vi "RemoteVI Status Convert.vi"(0 "raw":T2(array[cluster]), 1 "now":dbl) -> (4 "status":T1(array[cluster]))   [LabVIEW 2020, in "RemoteVI.lvlib"]
doc: "Turns the entries of RemoteVI Status Registry.vi into the status RemoteVI Status.vi returns, for the time now (seconds since the LabVIEW epoch): running is TRUE while the server loop published within the last 2 s; uptime s = now - started; per client connected s = now - since and idle s = now - last input, or -1 when the client sent no input yet; kB per s = bytes per s / 1024; hWnd (the shared window) is passed on. Pure function, cannot fail. Reference: statusConvert() in tools\\lib\\status.mjs, vectors tests\\vectors\\status.json (convert)."
uses:
  RemoteVI.lvlib
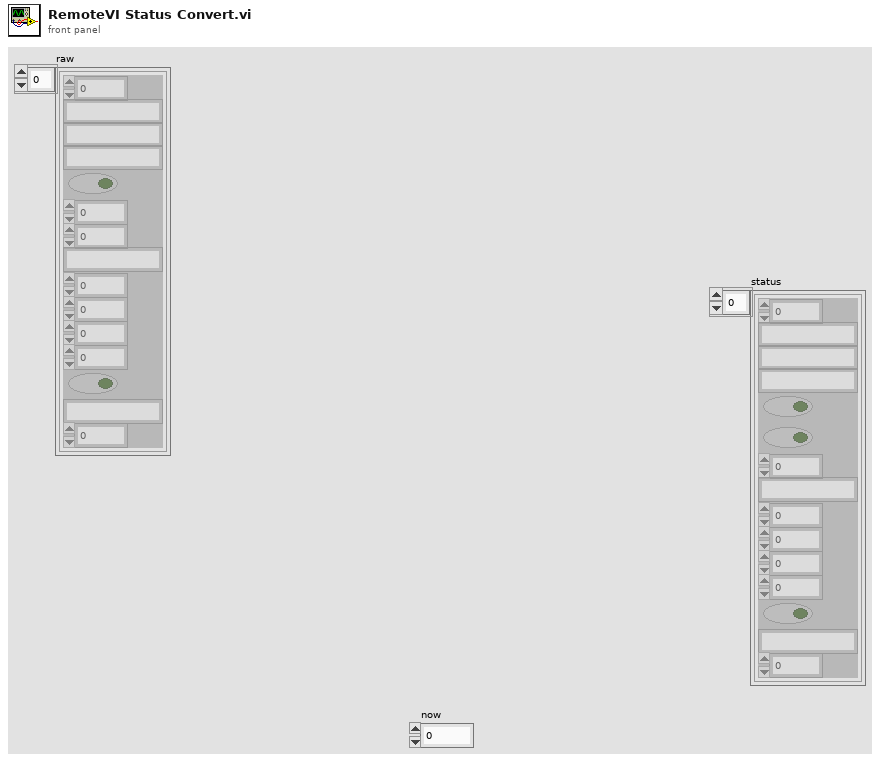
[diagram p1: front panel]
types:
  T1 = cluster{"port":u16, "url":string, "target":string, "kind":string, "whole network":bool, "running":bool, "uptime s":dbl, "clients":cluster{"address":string, "connected s":dbl, "idle s":dbl}[], "fps":dbl, "kB per s":dbl, "frames":u32, "latency ms":dbl, "view only":bool, "last error":string, "hWnd":u64}[]
  T2 = cluster{"port":u16, "url":string, "target":string, "kind":string, "whole network":bool, "started":dbl, "updated":dbl, "clients":cluster{"address":string, "since":dbl, "last input":dbl}[], "fps":dbl, "bytes per s":dbl, "frames":u32, "latency ms":dbl, "view only":bool, "last error":string, "hWnd":u64}[]
  T3 = cluster{"address":string, "connected s":dbl, "idle s":dbl}
  T4 = cluster{"port":u16, "url":string, "target":string, "kind":string, "whole network":bool, "running":bool, "uptime s":dbl, "clients":cluster{"address":string, "connected s":dbl, "idle s":dbl}[], "fps":dbl, "kB per s":dbl, "frames":u32, "latency ms":dbl, "view only":bool, "last error":string, "hWnd":u64}
  T5 = cluster{"address":string, "since":dbl, "last input":dbl}[]
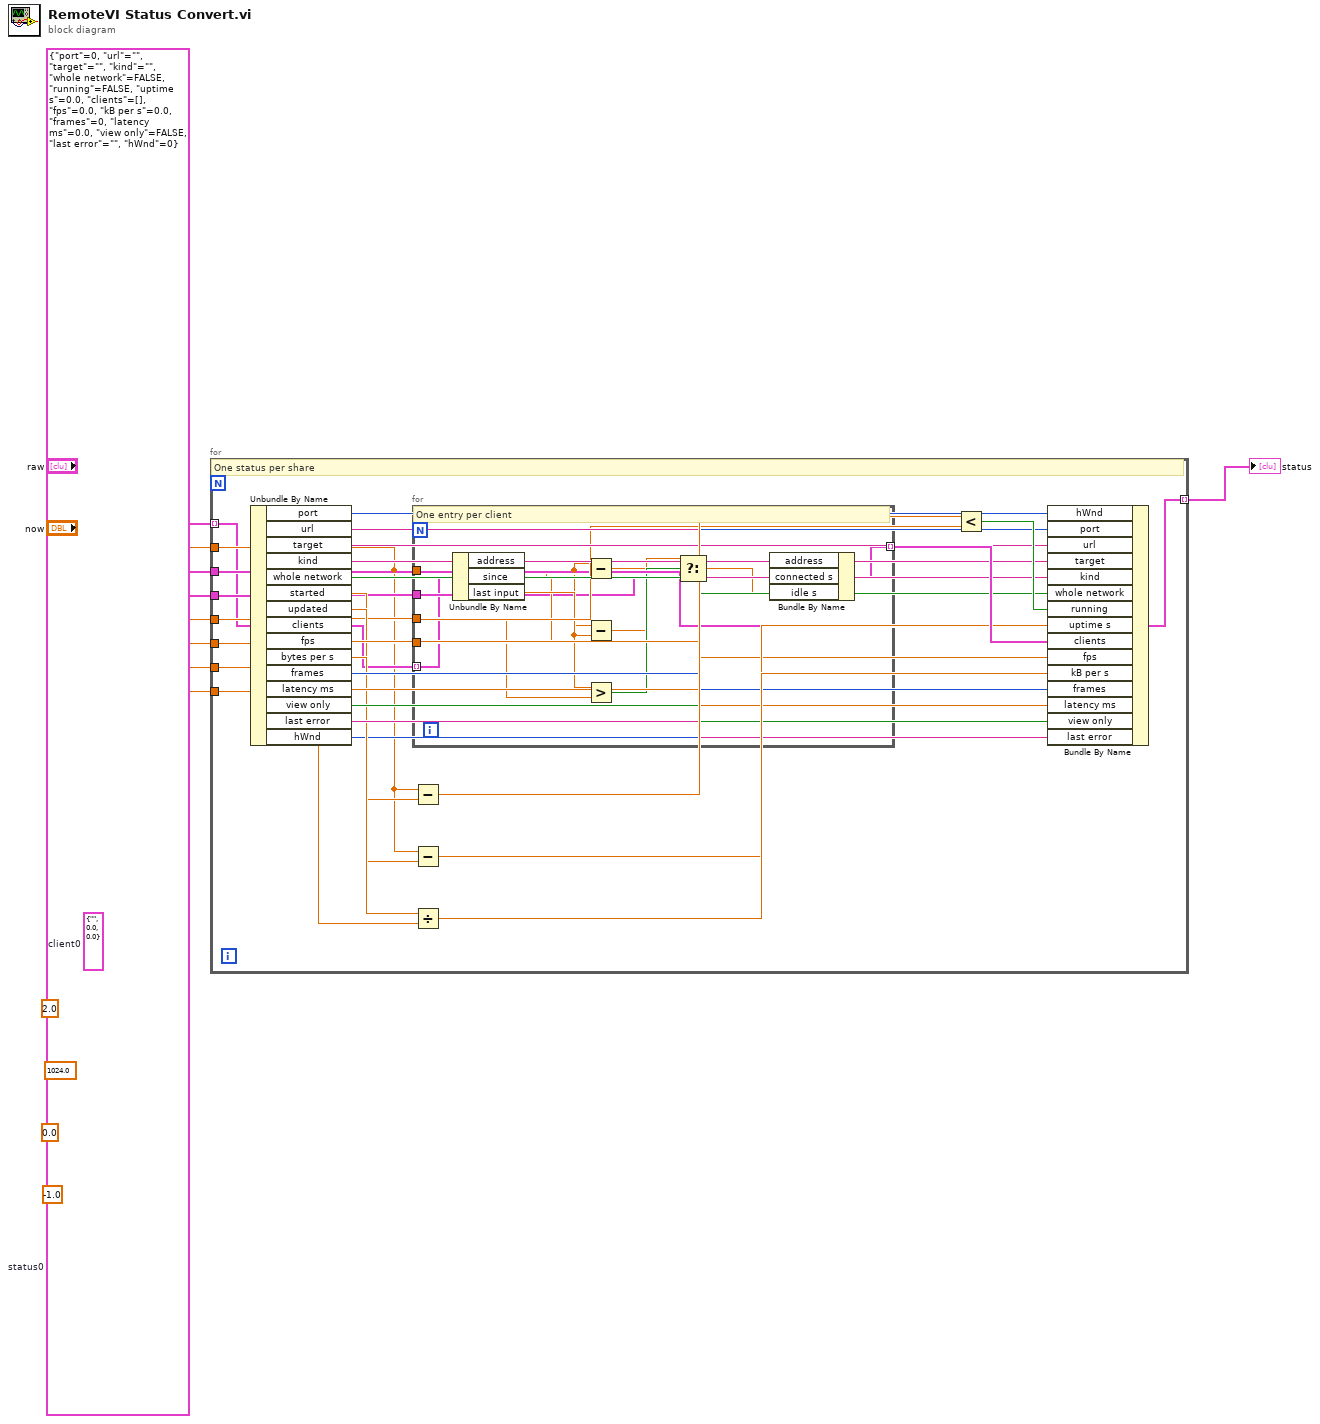
[diagram p0: block diagram]
diagram:
  w4 = T3 {"address"="", "connected s"=0.0, "idle s"=0.0}  # client0
  w3 = T4 {"port"=0, "url"="", "target"="", "kind"="", "whole network"=FALSE, "running"=FALSE, "uptime s"=0.0, "clients"=[], "fps"=0.0, "kB per s"=0.0, "frames"=0, "latency ms"=0.0, "view only"=FALSE, "last error"="", "hWnd"=0}  # status0
  n1 = for {
    tunnel: "raw" -> [w10] mode=indexing
    tunnel: "now" -> [w11]
    tunnel: w3 -> [w12]
    tunnel: w4 -> [w13]
    tunnel: 2.0 -> [w14]
    tunnel: 1024.0 -> [w15]
    tunnel: 0.0 -> [w16]
    tunnel: -1.0 -> [w17]
    tunnel: [w38] -> w9 mode=indexing
    # "One status per share"
    n2 = Unbundle By Name(w10) -> ("port"=w19:u16, "url"=w20:string, "target"=w21:string, "kind"=w22:string, "whole network"=w23:bool, "started"=w24:dbl, "updated"=w25:dbl, "clients"=w26:T5, "fps"=w27:dbl, "bytes per s"=w28:dbl, "frames"=w29:u32, "latency ms"=w30:dbl, "view only"=w31:bool, "last error"=w32:string, "hWnd"=w18:u64)
    n3 = for {
      tunnel: w11 -> [w40]
      tunnel: w13 -> [w41]
      tunnel: w16 -> [w42]
      tunnel: w17 -> [w43]
      tunnel: w26 -> [w39] mode=indexing
      tunnel: [w51] -> w37 mode=indexing
      # "One entry per client"
      n4 = Unbundle By Name(w39) -> ("address"=w44:string, "since"=w45:dbl, "last input"=w46:dbl)
      n5 = Subtract(x=w40, y=w45) -> (x-y=w47:dbl)
      n6 = Subtract(x=w40, y=w46) -> (x-y=w48:dbl)
      n7 = Greater?(x=w46, y=w42) -> (0:w49:bool)
      n8 = Select(t=w48, s=w49, f=w43) -> (s? t:f=w50:dbl)
      n9 = Bundle By Name(cluster=w41, "address"=w44, "connected s"=w47, "idle s"=w50) -> (w51:T3)
    }
    n10 = Subtract(x=w11, y=w25) -> (x-y=w33:dbl)
    n11 = Subtract(x=w11, y=w24) -> (x-y=w35:dbl)
    n12 = Divide(x=w28, y=w15) -> (x/y=w36:dbl)
    n13 = Less?(x=w33, y=w14) -> (x < y?=w34:bool)
    n14 = Bundle By Name(cluster=w12, "hWnd"=w18, "port"=w19, "url"=w20, "target"=w21, "kind"=w22, "whole network"=w23, "running"=w34, "uptime s"=w35, "clients"=w37, "fps"=w27, "kB per s"=w36, "frames"=w29, "latency ms"=w30, "view only"=w31, "last error"=w32) -> (w38:T4)
  }
  "status" <- w9
